vi "Configure.vi"(8 "error in (no error)":errorcluster, 9 "Path":path, 10 "Interactive?":bool, 11 "Text Report In":refnum<class "Text Report.lvclass">) -> (0 "error out":errorcluster, 3 "Text Report Out":refnum<class "Text Report.lvclass">)   [LabVIEW 2020, in "Text Report.lvclass"]
uses:
  Text Report.lvclass
  Text Report.lvclass/Text Report.ctl
  Framework/Configuration Manager/Configuration Manager.lvclass
panel:
  in  "Cancel":bool
  in  "Commit":bool
  in  "Open New Reports":bool
  in  "Report Path":path
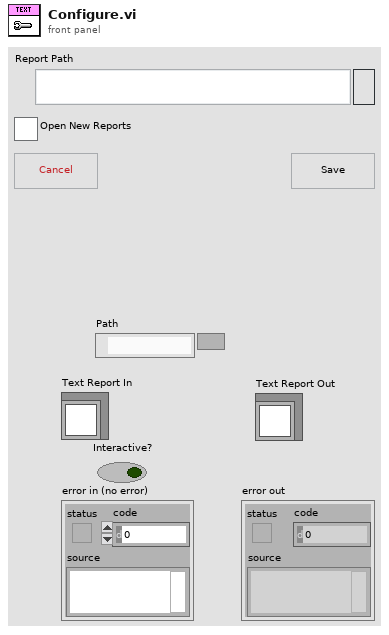
[diagram p1: front panel]
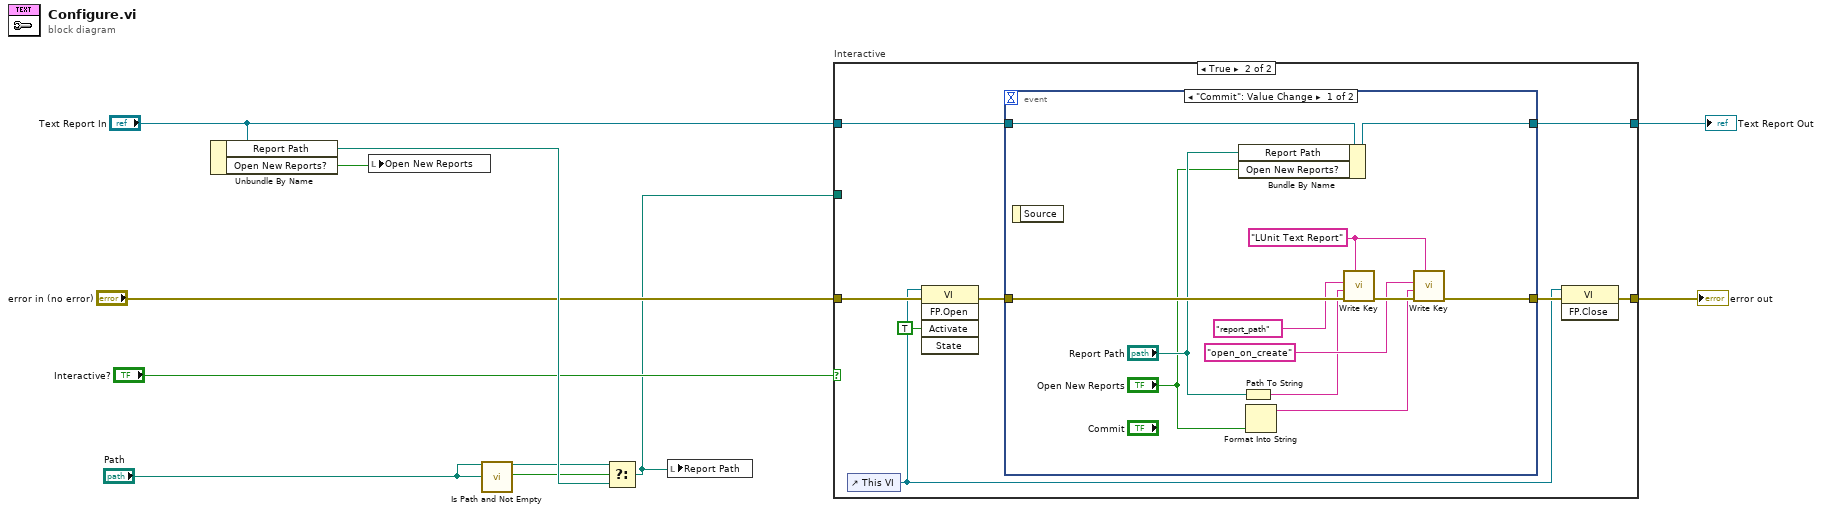
[diagram p0: block diagram]
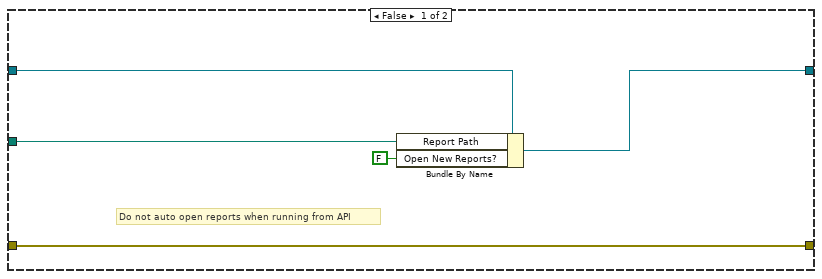
[diagram p2: hidden frame]
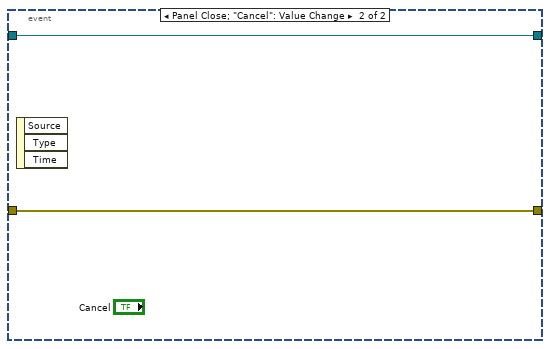
[diagram p3: hidden frame]
diagram:
  n1 = Unbundle By Name("Text Report In") -> ("Report Path"=w10:path, "Open New Reports?"=w1:bool)
  n2 = local write "Open New Reports"(w1) -> ()
  n3 = call <vilib>:"Is Path and Not Empty.vi"("path"="Path") -> ("Is Path and Not Empty?"=w3:bool)  [unwired: 4 in]
  n4 = Select(t="Path", s=w3, f=w10) -> (s? t:f=w4:path)
  n5 = local write "Report Path"(w4) -> ()
  n6 = case "Interactive" shown="True" "Interactive?" {
    tunnel: "error in (no error)" -> [w15 w21]
    tunnel: [w15 w19] -> w8
    tunnel: "Text Report In" -> [w14 w16]
    tunnel: [w13 w17] -> w6
    tunnel: w4 -> [w12 _]
    frame False {
      # "Do not auto open reports when running from API"
      n7 = Bundle By Name(cluster=w14, "Report Path"=w12, "Open New Reports?"=FALSE) -> (w13:refnum<class "Text Report.lvclass">)
    }
    frame True {
      n8 = control-ref of="This VI"() -> (w18:refnum<vi>)
      n9 = invoke class="VI" method="FP.Open"(reference=w18, error in=w21, "Activate"=TRUE ("Activate?")) -> (error out=w22:errorcluster)  [unwired: 2 in, 4 out]
      n10 = event shown="[0] \"Commit\": Value Change" {
        selector: _ -> [_ _]
        dyn-events: _ -> [_ _]
        timeout: _ -> [_ _]
        tunnel: w22 -> [w35 w37]
        tunnel: [w34 w37] -> w20
        tunnel: [w26 w36] -> w17
        tunnel: w16 -> [w27 w36]
        event "Commit": Value Change {
          w33 = "LUnit Text Report"
          n11 = event-data() -> ()  [unwired: 1 in, 1 out]
          n12 = Bundle By Name(cluster=w27, "Report Path"="Report Path", "Open New Reports?"="Open New Reports") -> (w26:refnum<class "Text Report.lvclass">)
          n13 = Path To String(path="Report Path") -> (string=w29:string)
          n14 = Format Into String("Open New Reports") -> (resulting string=w28:string)  [unwired: 3 in, 1 out]
          n15 = call "Write Key.vi"("section"=w33, "error in (no error)"=w35, "value"=w29, "key"="report_path" ("Name")) -> ("error out"=w32:errorcluster)  [unwired: 7 in]
          n16 = call "Write Key.vi"("section"=w33, "error in (no error)"=w32, "value"=w28, "key"="open_on_create" ("Name")) -> ("error out"=w34:errorcluster)  [unwired: 7 in]
        }
        event Panel Close; "Cancel": Value Change {
          n17 = event-data() -> ()  [unwired: 1 in, 3 out]
        }
      }
      n18 = invoke class="VI" method="FP.Close"(reference=w18, error in=w20) -> (error out=w19:errorcluster)  [unwired: 1 in, 2 out]
    }
  }
  "error out" <- w8
  "Text Report Out" <- w6
